vi "OwnOop20261013_ParentIsNoneV3.vi"() -> ()   [LabVIEW 2024]
panel:
  out "error out":errorcluster caption="错误输出"
  out "No Parent":bool
  in  "Class Path":path
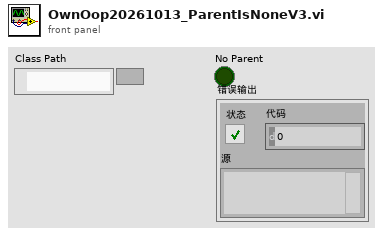
[diagram p1: front panel]
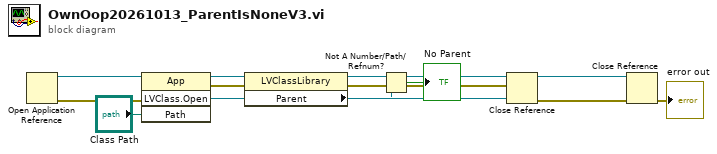
[diagram p0: block diagram]
diagram:
  n1 = Open Application Reference() -> (0:w8:errorcluster, 3:w10:refnum<vi>)  [unwired: 4 in]
  n2 = invoke class="App" method="LVClass.Open"(reference=w10, error in=w8, "Path"="Class Path") -> (error out=w6:errorcluster, "LVClass.Open"=w7:refnum<vi>)  [unwired: 1 in, 2 out]
  n3 = property class="LVClassLibrary"(reference=w7, error in=w6) -> (error out=w3:errorcluster, "Parent"=w5:refnum<vi>)  [unwired: 1 out]
  n4 = Not A Number/Path/Refnum?(number/path/refnum=w5) -> (NaN/Path/Refnum?=→"No Parent":bool)
  n5 = Close Reference(reference=w7, error in (no error)=w3) -> (error out=w2:errorcluster)
  n6 = Close Reference(reference=w10, error in (no error)=w2) -> (error out=→"error out":errorcluster)
